vi "Bundle Typed Base Probe.vi"() -> ()   [LabVIEW 2026]
doc: "Stage 2b: Bundle with a TYPED empty cluster constant as base (cluster: terminal) plus 3 element: inputs. Tests whether a typed-empty base (value=\"\") allows building a fresh 3-element cluster. Expected: Bundle Out={1,two,3.5}."
panel:
  out "Bundle Out":cluster{i32, string, dbl}={0, "\"\"", 0.0}
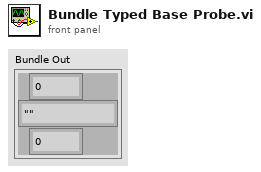
[diagram p1: front panel]
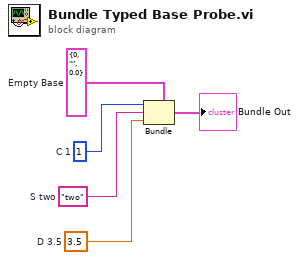
[diagram p0: block diagram]
diagram:
  w5 = cluster{i32, string, dbl} {0, "", 0.0}  # Empty Base
  w2 = 3.5  # D 3.5
  w3 = "two"  # S two
  w4 = 1  # C 1
  n1 = Bundle(cluster=w5, w4, w3, w2) -> (→"Bundle Out":cluster{i32, string, dbl})
